vi "Test_C_CIF.vi"() -> ()   [LabVIEW 2021]
uses:
  CANsub_C.lvlib
  C_RX_State.ctl
  api/CANsub_Channel/CANsub_Channel.lvclass
  api/CANsub_API.lvlib
  <vilib>/CIF Foundation/CIF PCAP Parse and Build/pcap_Parse_Build_CIF.lvclass
  <vilib>/CIF Foundation/CIF PCAP Parse and Build/Typedef/Time Format.ctl
  <vilib>/CIF Foundation/CIF Utilities/DataTypes/Typedef/Endian.ctl
  <vilib>/CIF Foundation/CIF Utilities/DataTypes/DataTypes_CIF_U.lvlib
  <vilib>/CIF Foundation/CIF PCAP Parse and Build/Typedef/File Format.ctl
  api/Pcap/CANsub_Pcap_Options.ctl
  api/Pcap/CANsub_Pcap_Results.ctl
  C_CIF_Encode_Result.ctl
  <vilib>/CIF Foundation/CIF PCAP Parse and Build/Typedef/Format Specific/CAN Interface Mode.ctl
  <vilib>/CIF Foundation/CIF PCAP Parse and Build/Typedef/Format Specific/CAN Metadata.ctl
panel:
  out "NI error out":errorcluster
  out "NI payloads":u8[][](array[numeric]) format="%.0x"
  out "NI metadata":T1[](array[typedef]) {"identifier" format="%.0x"}
  out "pass":bool
  out "stream length":i32
  out "encode result":T3
  in  "encode little endian":bool
  in  "tx size":i32=1740
  out "error out":errorcluster
  out "frames decoded":i32
  out "pcap bytes":u8[](array[numeric]) format="%02x"
  out "result":T4
  in  "options":T5={"allow list"=[], "deny list"=[], "TAI minus UTC (s)"=37, "keep TX acks"=FALSE, "little endian"=FALSE} {"deny list" format="%.0x"; "allow list" format="%.0x"}
  in  "max packets":i32=1756
  in  "first":i32
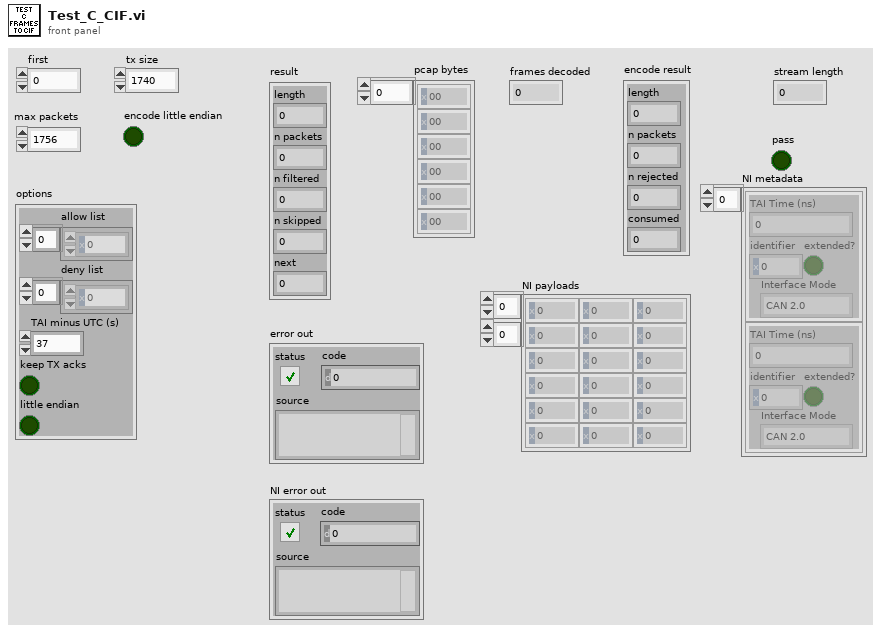
[diagram p1: front panel]
types:
  T1 = typedef "pcap_Parse_Build_CIF.lvclass/CAN Metadata.ctl" = cluster{"TAI Time (ns)":i64, "identifier":u32, "extended?":bool, "Interface Mode":T2}
  T2 = typedef "pcap_Parse_Build_CIF.lvclass/CAN Interface Mode.ctl" = enum16{"CAN 2.0", "CAN FD", "CAN FD BRS", "Remote"}
  T3 = typedef "CANsub_C.lvlib/C_CIF_Encode_Result.ctl" = cluster{"length":i32, "n packets":i32, "n rejected":i32, "consumed":i32}
  T4 = typedef "CANsub_API.lvlib/CANsub_Pcap_Results.ctl" = cluster{"length":i32, "n packets":i32, "n filtered":i32, "n skipped":i32, "next":i32}
  T5 = typedef "CANsub_API.lvlib/CANsub_Pcap_Options.ctl" = cluster{"allow list":u32[], "deny list":u32[], "TAI minus UTC (s)":i32, "keep TX acks":bool, "little endian":bool}
  T6 = typedef "DataTypes_CIF_U.lvlib/Endian.ctl" = enum16{"Little Endian", "Big Endian"}
  T7 = typedef "pcap_Parse_Build_CIF.lvclass/File Format.ctl" = cluster{"Endian":T6, "Time Format":T8}
  T8 = typedef "pcap_Parse_Build_CIF.lvclass/Time Format.ctl" = enum16{"us", "ns"}
  T9 = typedef "CANsub_C.lvlib/C_RX_State.ctl" = cluster{"ws":u8[], "hdlc":u8[], "ping":u8[]}
  T10 = typedef "CANsub_C.lvlib/C_RX_Buffers.ctl" = cluster{"t_dev":dbl[], "ws":u8[], "id":u32[], "flags":u16[], "hdlc":u8[], "dlc":u8[], "data len":u8[], "data":u8[], "ping":u8[]}
  T11 = typedef "CANsub_API.lvlib/CANsub_Frames.ctl" = cluster{"count":i32, "t_dev":dbl[], "id":u32[], "flags":u16[], "dlc":u8[], "data len":u8[], "data":u8[]}
  T12 = typedef "CANsub_C.lvlib/C_Decode_Result.ctl" = cluster{"n frames":i32, "peer close":bool, "ping len":i32, "crc errors":u32, "decode errors":i32}
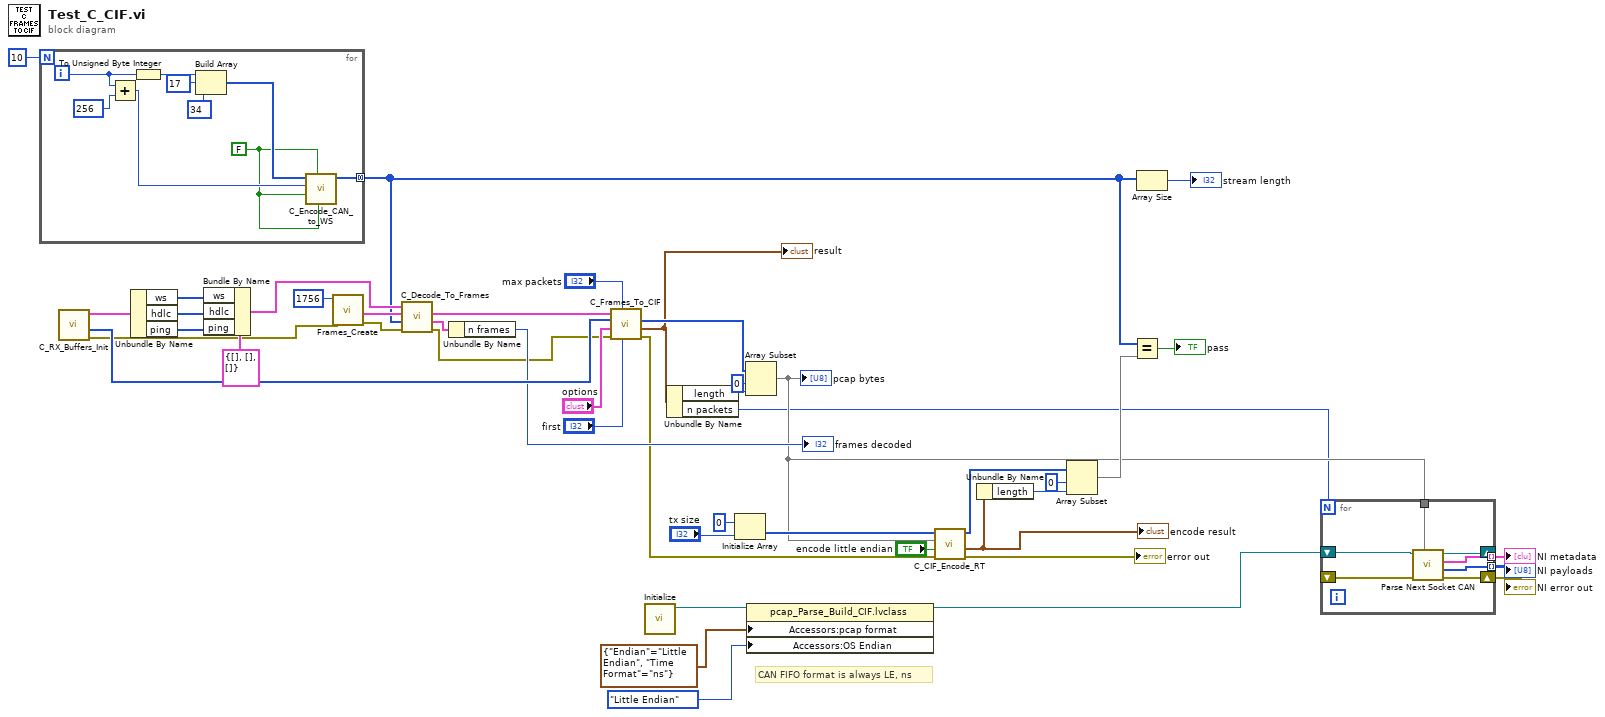
[diagram p0: block diagram]
diagram:
  # "CAN FIFO format is always LE, ns"
  n1 = for {
    N: 10 -> [_]
    tunnel: [w50] -> w12 mode=concatenating
    i -> [w53]
    w47 = FALSE ("ide")
    n2 = Add(x=w53, y=u32 256) -> (x+y=w49:u32)
    n3 = To Unsigned Byte Integer(number=w53) -> (unsigned 8bit integer=w54:u8)
    n4 = Build Array(w54, u8 17 ("element"), u8 34 ("element")) -> (w48:u8[])
    n5 = call "C_Encode_CAN_to_WS.vi"("brs"=w47, "ide"=w47, "fdf"=w47, "id"=w49, "data"=w48) -> ("ws frame"=w50:u8[])  [unwired: 5 in, 1 out]
  }
  n6 = call "C_RX_Buffers_Init.vi"() -> ("error out"=w25:errorcluster, "pcap"=w35:u8[], "buffers"=w44:T10)  [unwired: 8 in, 1 out]
  n7 = Unbundle By Name(w44) -> ("ws"=w43:u8[], "hdlc"=w42:u8[], "ping"=w41:u8[])
  n8 = Bundle By Name(cluster=T9 {"ws"=[], "hdlc"=[], "ping"=[]} ("C_RX_State"), "ws"=w43, "hdlc"=w42, "ping"=w41) -> (w38:T9)
  n9 = call "Frames_Create.vi"("error in (no error)"=w25, "capacity"=1756) -> ("error out"=w24:errorcluster, "frames"=w39:T11)  [unwired: 8 in]
  n10 = call "C_Decode_To_Frames.vi"("error in (no error)"=w24, "bytes in"=w12, "frames in"=w39, "state in"=w38) -> ("error out"=w26:errorcluster, "result"=w37:T12, "frames out"=w36:T11)  [unwired: 4 in, 1 out]
  n11 = Unbundle By Name(w37) -> ("n frames"=→"frames decoded":i32)
  n12 = call "C_Frames_To_CIF.vi"("first"="first", "max packets"="max packets", "error in (no error)"=w26, "options"="options", "pcap in"=w35, "frames in"=w36) -> ("error out"=w19:errorcluster, "result"=w28:T4, "pcap out"=w31:u8[])  [unwired: 2 in, 1 out]
  "result" <- w28
  n13 = call <vilib>:"Initialize.vi"() -> ("pcap Parse and Build out"=w9:refnum<class "pcap_Parse_Build_CIF.lvclass">)  [unwired: 11 in]
  n14 = Unbundle By Name(w28) -> ("length"=w30:i32, "n packets"=w1:i32)
  n15 = Initialize Array(u8 0 ("element"), "tx size") -> (w21:u8[])
  n16 = Array Subset(array=w31, index=0, length=w30) -> (w2:u8[])
  "pcap bytes" <- w2
  n17 = property class="pcap_Parse_Build_CIF.lvclass"(reference=w9, "Accessors:pcap format"=T7 {"Endian"=enum."Little Endian", "Time Format"=enum."ns"} ("pcap format"), "Accessors:OS Endian"=Endian."Little Endian" ("OS Endian")) -> (reference out=w7:refnum<class "pcap_Parse_Build_CIF.lvclass">)  [unwired: 1 in, 1 out]
  n18 = call "C_CIF_Encode_RT.vi"("error in (no error)"=w19, "little endian"="encode little endian", "pcap"=w2, "tx in"=w21) -> ("error out"=→"error out":errorcluster, "result"=w17:T3, "tx out"=w15:u8[])  [unwired: 5 in]
  "encode result" <- w17
  n19 = Unbundle By Name(w17) -> ("length"=w16:i32)
  n20 = Array Subset(array=w15, index=0, length=w16) -> (w6:u8[])
  n21 = Equal?(x=w12, y=w6) -> (x = y?=→"pass":bool)
  n22 = Array Size(array=w12) -> (size(s)=→"stream length":i32)
  n23 = for {
    N: w1 -> [_]
    shift-right: [w61] -> _
    shift-left: w7 -> [w62]
    tunnel: w2 -> [w60]
    shift-right: [w59] -> w3
    shift-left: _ -> [w58]
    tunnel: [w57] -> w5 mode=indexing
    tunnel: [w56] -> w4 mode=indexing
    n24 = call <vilib>:"Parse Next Socket CAN.vi"("CAN pcap in"=w60, "error in (no error)"=w58, "pcap Parse and Build in"=w62) -> ("error out"=w59:errorcluster, "Payload"=w56:u8[], "CAN Metadata"=w57:T1, "pcap Parse and Build out"=w61:refnum<class "pcap_Parse_Build_CIF.lvclass">)  [unwired: 4 in, 1 out]
  }
  "NI metadata" <- w5
  "NI payloads" <- w4
  "NI error out" <- w3
